vi "DAC Save Results.vi"(8 "error in":errorcluster, 9 "Log Details?":bool, 10 "tdms file":refnum<k34>, 11 "DAC ADV in":refnum<class "DAC ADV.lvclass">) -> (0 "error out":errorcluster)   [LabVIEW 2019, in "DAC.lvlib" / "DAC ADV.lvclass"]
uses:
  DAC ADV.lvclass
  C:/Users/krio/Documents/LV_Projects/test-stand/App/DAC/DAC.lvclass
  DAC.lvclass/DAC.ctl
  DAC ADV.lvclass/DAC ADV.ctl
  DAC.lvclass
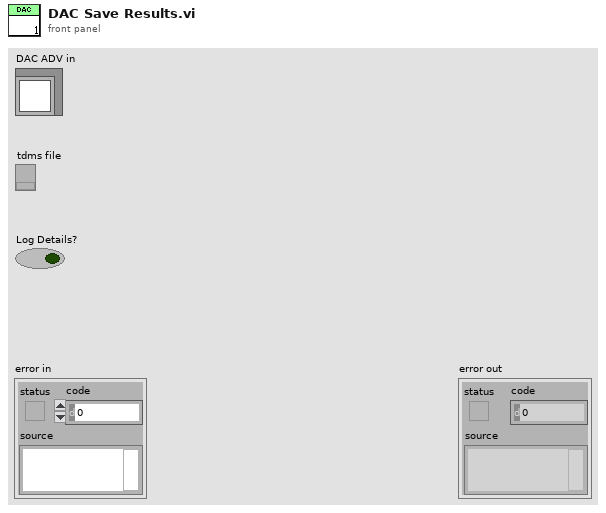
[diagram p1: front panel]
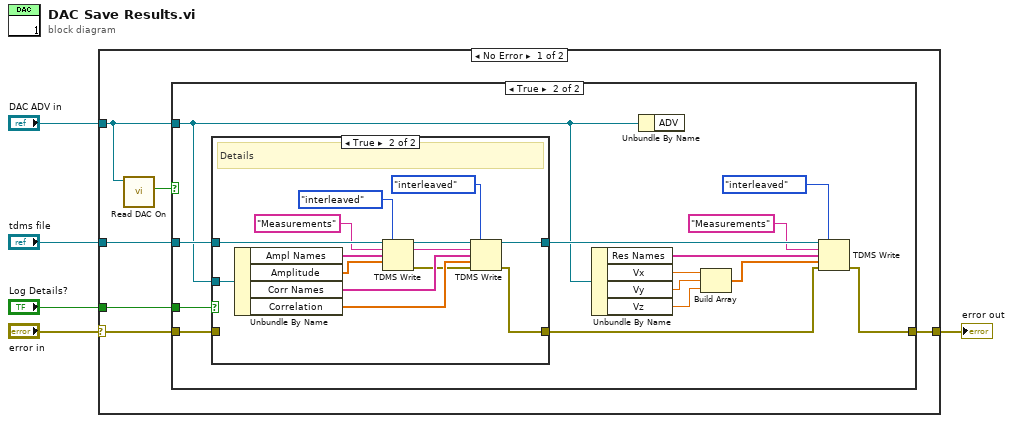
[diagram p0: block diagram]
diagram:
  n1 = case shown="No Error" "error in" {
    selector: "error in" -> [w6 w43]
    tunnel: "DAC ADV in" -> [w11 _]
    tunnel: "tdms file" -> [w9 _]
    tunnel: [w8 w43] -> w2
    tunnel: "Log Details?" -> [w7 _]
    frame No Error {
      n2 = call "Read DAC On.vi"("DAC in"=w11) -> ("DAC On"=w10:bool)  [unwired: 8 in, 2 out]
      n3 = case shown="True" w10 {
        tunnel: w11 -> [_ w21]
        tunnel: w9 -> [_ w24]
        tunnel: [w12 w26] -> w8
        tunnel: w7 -> [_ w25]
        tunnel: w6 -> [w12 w15]
        frame False {
        }
        frame True {
          n4 = case shown="True" w25 {
            tunnel: w24 -> [w28 w42]
            tunnel: [w28 w36] -> w23
            tunnel: w21 -> [_ w41]
            tunnel: w15 -> [w27 _]
            tunnel: [w27 w31] -> w14
            frame False {
            }
            frame True {
              # "Details"
              n5 = Unbundle By Name(w41) -> ("Ampl Names"=w40:string[], "Amplitude"=w38:dbl[], "Corr Names"=w34:string[], "Correlation"=w33:dbl[])
              n6 = TDMS Write(0:w42, 1:enum16{"decimated", "interleaved"}."interleaved" ("data layout (0:decimated)"), 5:"Measurements" ("group name in (Untitled)"), 7:w40, 9:w38) -> (4:w37:refnum<k34>, 6:w35:string, 15:w32:errorcluster)  [unwired: 1 in, 1 out]
              n7 = TDMS Write(0:w37, 1:enum16{"decimated", "interleaved"}."interleaved" ("data layout (0:decimated)"), 5:w35, 7:w34, 9:w33, 11:w32) -> (4:w36:refnum<k34>, 15:w31:errorcluster)  [unwired: 2 out]
            }
          }
          n8 = Unbundle By Name(w21) -> ("Res Names"=w17:string[], "Vx"=w20:dbl, "Vy"=w19:dbl, "Vz"=w18:dbl)
          n9 = Unbundle By Name(w21) -> ()  [unwired: 1 out]
          n10 = Build Array(w20, w19, w18) -> (w16:dbl[])
          n11 = TDMS Write(0:w23, 1:enum16{"decimated", "interleaved"}."interleaved" ("data layout (0:decimated)"), 5:"Measurements" ("group name in (Untitled)"), 7:w17, 9:w16, 11:w14) -> (15:w26:errorcluster)  [unwired: 3 out]
        }
      }
    }
    frame Error {
    }
  }
  "error out" <- w2
